vi "Enemy_Climb.vi"(0 "Tiles":u8[][](array[numeric]), 5 "Enemy":T1={"Kind"=0, "X10"=0, "Y10"=0, "Dir"=1, "Mode"=0}, 7 "Speed":i32, 9 "Random":i32, 11 "error in":errorcluster) -> (4 "Y10":i32, 6 "Dir":i32, 8 "Mode":i32, 15 "error out":errorcluster)   [LabVIEW 2020, in "GH_Engine.lvlib"]
doc: "One step of a climbing spider: up or down; on reaching a floor or the top it walks on in a random direction (Random), at the end of a rope or the top of the room it turns. Inline subVI of Enemies_Step."
uses:
  GH_Engine.lvlib
  Level/GH_Level.lvlib
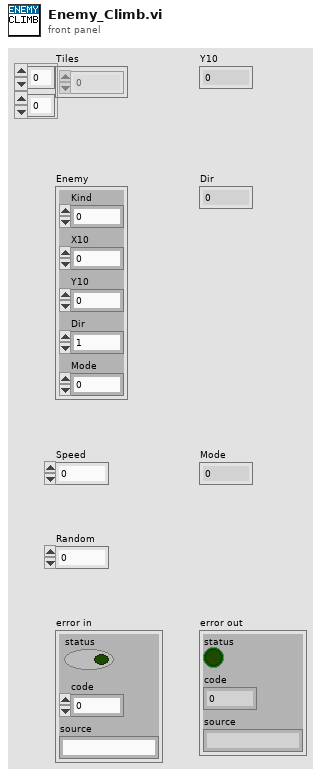
[diagram p1: front panel]
types:
  T1 = cluster{"Kind":i32, "X10":i32, "Y10":i32, "Dir":i32, "Mode":i32}
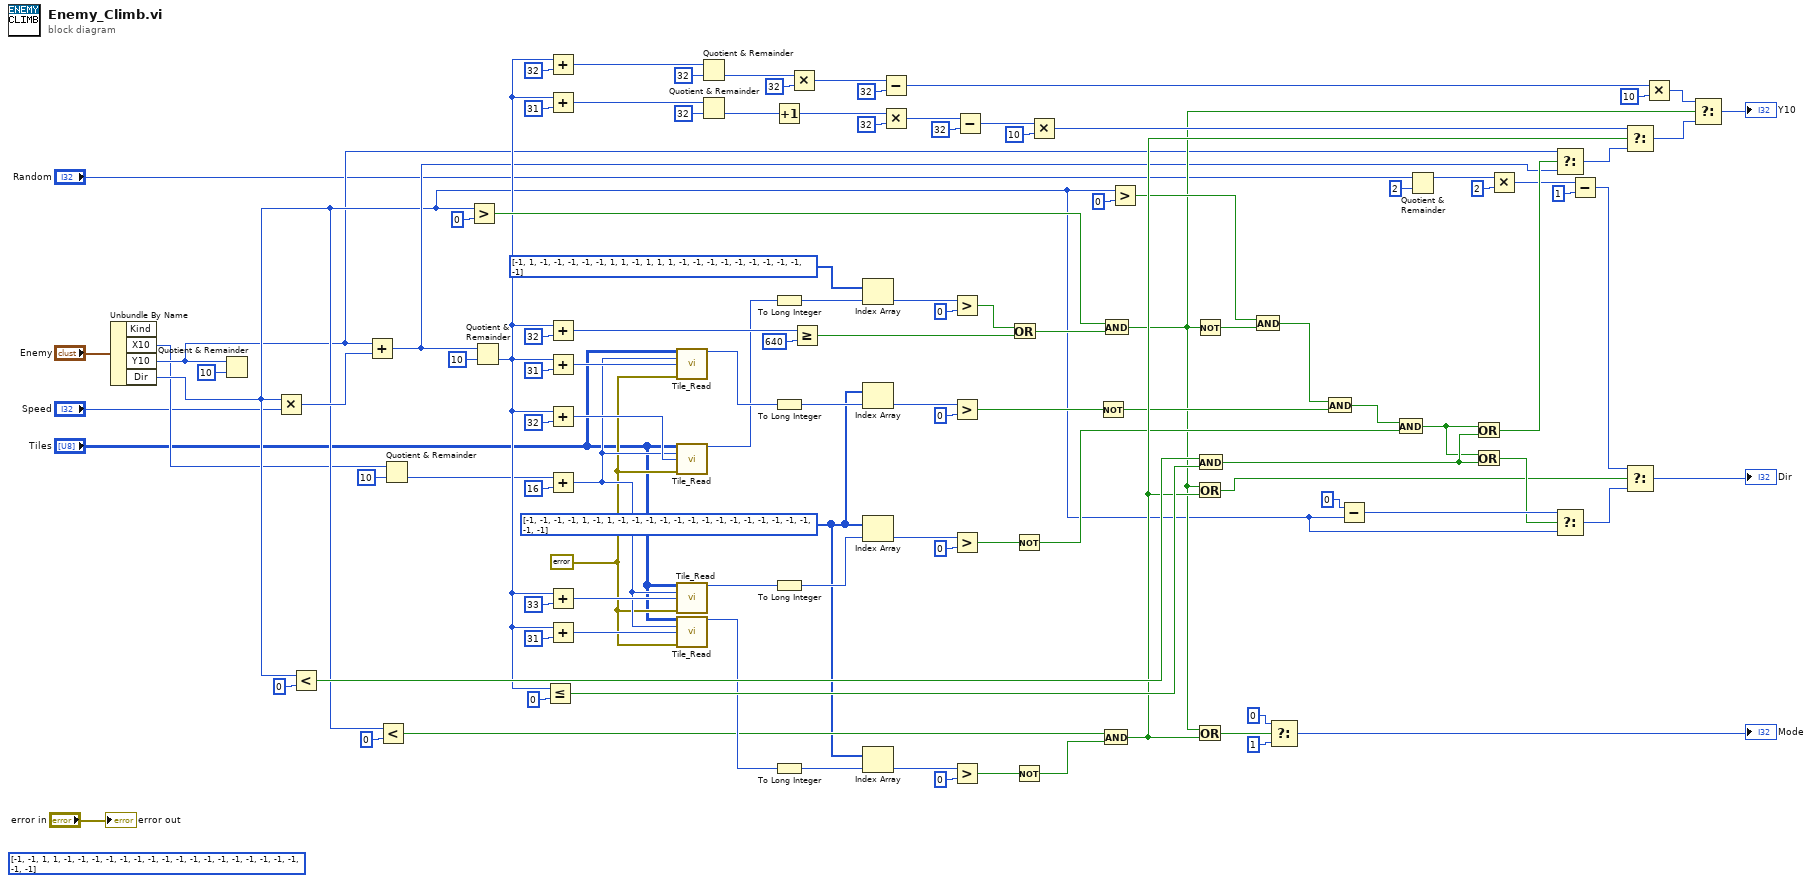
[diagram p0: block diagram]
diagram:
  w11 = errorcluster {"status"=FALSE, "code"=0, "source"=""} ("no error")
  w7 = i32[] [-1, -1, -1, -1, 1, -1, 1, -1, -1, -1, -1, -1, -1, -1, -1, -1, -1, -1, -1, -1, -1, -1, -1] ("Ladder or rope")
  (unwired) i32[] [-1, -1, 1, 1, -1, -1, -1, -1, -1, -1, -1, -1, -1, -1, -1, -1, -1, -1, -1, -1, -1, -1, -1] ("Thin floor")
  n1 = Unbundle By Name("Enemy") -> ("X10"=w8:i32, "Y10"=w9:i32, "Dir"=w10:i32)  [unwired: 1 out]
  n2 = Quotient & Remainder(x=w9, y=10) -> ()  [unwired: 2 out]
  n3 = Multiply(x=w10, y="Speed") -> (x*y=w15:i32)
  n4 = Less?(x=w10, y=0) -> (x < y?=w93:bool)
  n5 = Add(x=w9, y=w15) -> (x+y=w16:i32)
  n6 = Less?(x=w10, y=0) -> (x < y?=w73:bool)
  n7 = Quotient & Remainder(x=w8, y=10) -> (floor(x/y)=w13:i32)  [unwired: 1 out]
  n8 = Greater?(x=w10, y=0) -> (0:w28:bool)
  n9 = Quotient & Remainder(x=w16, y=10) -> (floor(x/y)=w18:i32)  [unwired: 1 out]
  n10 = Less Or Equal?(x=w18, y=0) -> (x <= y?=w95:bool)
  n11 = Add(x=w18, y=32) -> (x+y=w43:i32)
  n12 = Add(x=w18, y=31) -> (x+y=w84:i32)
  n13 = Add(x=w18, y=32) -> (x+y=w37:i32)
  n14 = Add(x=w18, y=31) -> (x+y=w54:i32)
  n15 = Add(x=w18, y=32) -> (x+y=w30:i32)
  n16 = Add(x=w13, y=16) -> (x+y=w20:i32)
  n17 = Add(x=w18, y=33) -> (x+y=w62:i32)
  n18 = Add(x=w18, y=31) -> (x+y=w75:i32)
  n19 = call "Tile_Read.vi"("Tiles"="Tiles", "X"=w20, "Y"=w54, "error in"=w11) -> ("Tile"=w55:u8)  [unwired: 10 in, 1 out]
  n20 = call "Tile_Read.vi"("Tiles"="Tiles", "X"=w20, "Y"=w30, "error in"=w11) -> ("Tile"=w31:u8)  [unwired: 10 in, 1 out]
  n21 = call "Tile_Read.vi"("Tiles"="Tiles", "X"=w20, "Y"=w62, "error in"=w11) -> ("Tile"=w63:u8)  [unwired: 10 in, 1 out]
  n22 = call "Tile_Read.vi"("Tiles"="Tiles", "X"=w20, "Y"=w75, "error in"=w11) -> ("Tile"=w76:u8)  [unwired: 10 in, 1 out]
  n23 = Quotient & Remainder(x=w43, y=32) -> (floor(x/y)=w45:i32)  [unwired: 1 out]
  n24 = Quotient & Remainder(x=w84, y=32) -> (floor(x/y)=w86:i32)  [unwired: 1 out]
  n25 = Increment(x=w86) -> (x+1=w87:i32)
  n26 = To Long Integer(number=w31) -> (32bit integer=w32:i32)
  n27 = To Long Integer(number=w55) -> (32bit integer=w56:i32)
  n28 = To Long Integer(number=w63) -> (32bit integer=w64:i32)
  n29 = To Long Integer(number=w76) -> (32bit integer=w77:i32)
  n30 = Multiply(x=w45, y=32) -> (x*y=w47:i32)
  n31 = Greater Or Equal?(x=w37, y=640) -> (x >= y?=w39:bool)
  n32 = Index Array(array=i32[] [-1, 1, -1, -1, -1, -1, -1, 1, 1, -1, 1, 1, 1, -1, -1, -1, -1, -1, -1, -1, -1, -1, -1] ("Solid"), index=w32) -> (element=w33:i32)
  n33 = Index Array(array=w7, index=w56) -> (element=w57:i32)
  n34 = Index Array(array=w7, index=w64) -> (element=w65:i32)
  n35 = Index Array(array=w7, index=w77) -> (element=w78:i32)
  n36 = Subtract(x=w47, y=32) -> (x-y=w49:i32)
  n37 = Multiply(x=w87, y=32) -> (x*y=w89:i32)
  n38 = Greater?(x=w33, y=0) -> (0:w35:bool)
  n39 = Greater?(x=w57, y=0) -> (0:w59:bool)
  n40 = Greater?(x=w65, y=0) -> (0:w67:bool)
  n41 = Greater?(x=w78, y=0) -> (0:w80:bool)
  n42 = Subtract(x=w89, y=32) -> (x-y=w91:i32)
  n43 = Or(x=w35, y=w39) -> (x .or. y?=w40:bool)
  n44 = Not(x=w67) -> (.not. x?=w68:bool)
  n45 = Not(x=w80) -> (.not. x?=w81:bool)
  n46 = Multiply(x=w91, y=10) -> (x*y=w100:i32)
  n47 = Not(x=w59) -> (.not. x?=w60:bool)
  n48 = And(x=w73, y=w81) -> (x .and. y?=w82:bool)
  n49 = And(x=w28, y=w40) -> (x .and. y?=w41:bool)
  n50 = Greater?(x=w10, y=0) -> (0:w51:bool)
  n51 = Not(x=w41) -> (.not. x?=w52:bool)
  n52 = Or(x=w41, y=w82) -> (x .or. y?=w105:bool)
  n53 = Or(x=w41, y=w82) -> (x .or. y?=w111:bool)
  n54 = And(x=w93, y=w95) -> (x .and. y?=w96:bool)
  n55 = And(x=w51, y=w52) -> (x .and. y?=w69:bool)
  n56 = Select(t=0, s=w111, f=1) -> (s? t:f=→"Mode":i32)
  n57 = And(x=w69, y=w60) -> (x .and. y?=w70:bool)
  n58 = Subtract(x=0, y=w10) -> (x-y=w108:i32)
  n59 = And(x=w70, y=w68) -> (x .and. y?=w71:bool)
  n60 = Quotient & Remainder(x="Random", y=2) -> (x-y*floor(x/y)=w22:i32)  [unwired: 1 out]
  n61 = Or(x=w71, y=w96) -> (x .or. y?=w101:bool)
  n62 = Or(x=w71, y=w96) -> (x .or. y?=w106:bool)
  n63 = Multiply(x=w22, y=2) -> (x*y=w24:i32)
  n64 = Select(t=w9, s=w101, f=w16) -> (s? t:f=w102:i32)
  n65 = Select(t=w108, s=w106, f=w10) -> (s? t:f=w109:i32)
  n66 = Subtract(x=w24, y=1) -> (x-y=w26:i32)
  n67 = Select(t=w100, s=w82, f=w102) -> (s? t:f=w103:i32)
  n68 = Select(t=w26, s=w105, f=w109) -> (s? t:f=→"Dir":i32)
  n69 = Multiply(x=w49, y=10) -> (x*y=w98:i32)
  n70 = Select(t=w98, s=w41, f=w103) -> (s? t:f=→"Y10":i32)
  "error out" <- "error in"
